vi "PicoScope4000ExampleBlock.vi"() -> ()   [LabVIEW 2012]
doc: "This example demonstrates how to use the PicoScope Labview library to collect data using block mode."
uses:
  shared/PicoBuffers.ctl
  shared/Acquisition Settings.ctl
  PicoScope4000Lib/PicoScope4000AnalogChannelSettingsIEPE.ctl
  PicoScope4000Lib/PicoScope4000Buffer and Transfer Settings.ctl
panel:
  in  "Channel B Settings":T1={"Enabled"=TRUE, "Range"=6, "Bandwidth Limit"=0, "Coupling"=1} {"Coupling" items=["AC", "DC", "IEPE"]; "Bandwidth Limit" items=["Off", "200kHz"]; "Range" items=["10 mV", "20 mV", "50 mV", "100 mV", "200 mV", "500 mV", "1 V", "2 V", "5 V", "10 V", "20 V", "50 V ", "100 V"]}
  out "Unit Info":T2
  in  "PicoScope 4262 Ext. Trigger Range":u32(ring)=5 items=["500 mV"=5, "5 V"=8]
  in  "Trigger Settings":T3={"Trigger Enabled"=FALSE, "Trigger Source"=enum."Channel A", "Trigger Threshold (Volts)"=0.0, "Trigger Direction"=2, "Trigger Delay (samples)"=0, "Auto Trigger Time (ms)"=1000} {"Trigger Direction" items=["Rising"=2, "Falling"=3]}
  in  "Channel A Settings":T1={"Enabled"=TRUE, "Range"=6, "Bandwidth Limit"=0, "Coupling"=1} {"Coupling" items=["AC", "DC", "IEPE"]; "Bandwidth Limit" items=["Off", "200kHz"]; "Range" items=["10 mV", "20 mV", "50 mV", "100 mV", "200 mV", "500 mV", "1 V", "2 V", "5 V", "10 V", "20 V", "50 V ", "100 V"]}
  out "overflow":i16 format="%08b"
  in  "Apply Settings":bool
  out "error out":errorcluster
  in  "Data file":path=path "PicoScope4000ExampleBlock ChA Data"
  in  "Buffer and Transfer Settings":T4={"startIndex"=0, "Samples"=5000000, "Down Sample Ratio"=1, "Down-Sample Mode"=0} {"Down-Sample Mode" items=["None", "Aggregate", "Average"]; "Down Sample Ratio" step=1; "Samples" format="%_6p"}
  in  "Acquisition Settings":T5={"preTriggerSamples"=0, "postTriggerSamples"=5000000, "timebase"=5} {"postTriggerSamples" format="%_6p"; "preTriggerSamples" format="%_6p"}
  out "Properties Panel":T6 {"Max Total Capture Time Available (sec)" format="%.3p"; "Sample Frequency" format="%.6p"; "Sample Rate" format="%.3p"; "Max Samples Available" format="%_6p"; "Total Capture Time (sec)" format="%.3p"}
  in  "stop":bool
  out "Analog Channels":cluster{i32, dbl, "Data":dbl[]}[](graph)
  in  "Serial Number":string
  in  "Use Serial Number":bool
  in  "error in (no error)":errorcluster
  # "Bit 0 = ChA"
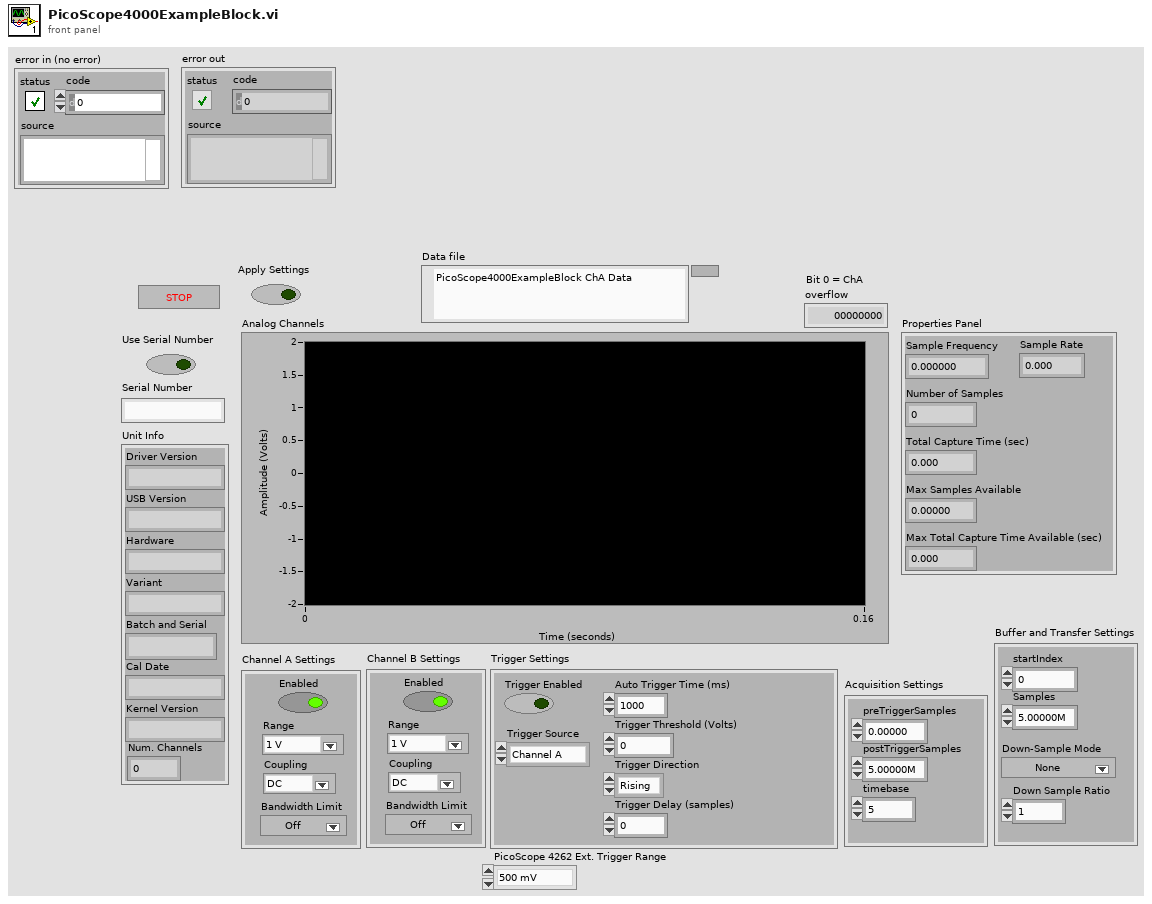
[diagram p1: front panel]
types:
  T1 = typedef "PicoScope4000AnalogChannelSettingsIEPE.ctl" = cluster{"Enabled":bool, "Range":u16, "Bandwidth Limit":i16, "Coupling":u16}
  T2 = cluster{"Driver Version":string, "USB Version":string, "Hardware":string, "Variant":string, "Batch and Serial":string, "Cal Date":string, "Kernel Version":string, "Num. Channels":i16}
  T3 = cluster{"Trigger Enabled":bool, "Trigger Source":enum16{"Channel A", "Channel B", "Channel C", "Channel D", "Channel E", "Channel F", "Channel G", "Channel H"}, "Trigger Threshold (Volts)":dbl, "Trigger Direction":u16, "Trigger Delay (samples)":u32, "Auto Trigger Time (ms)":i16}
  T4 = typedef "PicoScope4000Buffer and Transfer Settings.ctl" = cluster{"startIndex":u64, "Samples":u64, "Down Sample Ratio":u64, "Down-Sample Mode":u32}
  T5 = typedef "Acquisition Settings.ctl" = cluster{"preTriggerSamples":u64, "postTriggerSamples":u64, "timebase":u32}
  T6 = cluster{"Sample Frequency":dbl, "Sample Rate":dbl, "Max Samples Available":u64, "Number of Samples":u64, "Total Capture Time (sec) ":dbl, "Max Total Capture Time Available (sec)":dbl}
  T7 = enum16{"open", "open or create", "create or replace", "create", "open (read-only)"}
  T8 = typedef "PicoBuffers.ctl" = cluster{"Max Buffer Pointers":u64[][][], "Min Buffer Pointers":u64[][][], "StreamingDataInfo":cluster{"Channel":u32, "Down-Sample Mode":u32, "PICO_DATA_TYPE":enum32{"PICO_INT8_T", "PICO_INT16_T", "PICO_INT32_T", "PICO_UINT32_T", "PICO_INT64_T", ""}, "Samples":i32, "bufferIndex":u64, "startIndex":i32, "overflow":i16}[][]}
  T9 = cluster{"Channel A Buffer":i16[], "Channel B Buffer":i16[], "Channel C Buffer":i16[], "Channel D Buffer":i16[], "Channel E Buffer":i16[], "Channel F Buffer":i16[], "Channel G Buffer":i16[], "Channel H Buffer":i16[], "Port 0 Buffer":i16[], "Port 1 Buffer":i16[]}[]
  T10 = cluster{"Channel A Buffer":i16[], "Channel B Buffer":i16[], "Channel C Buffer":i16[], "Channel D Buffer":i16[], "Channel E Buffer":i16[], "Channel F Buffer":i16[], "Channel G Buffer":i16[], "Channel H Buffer":i16[], "Port 0 Buffer":i16[], "Port 1 Buffer":i16[]}
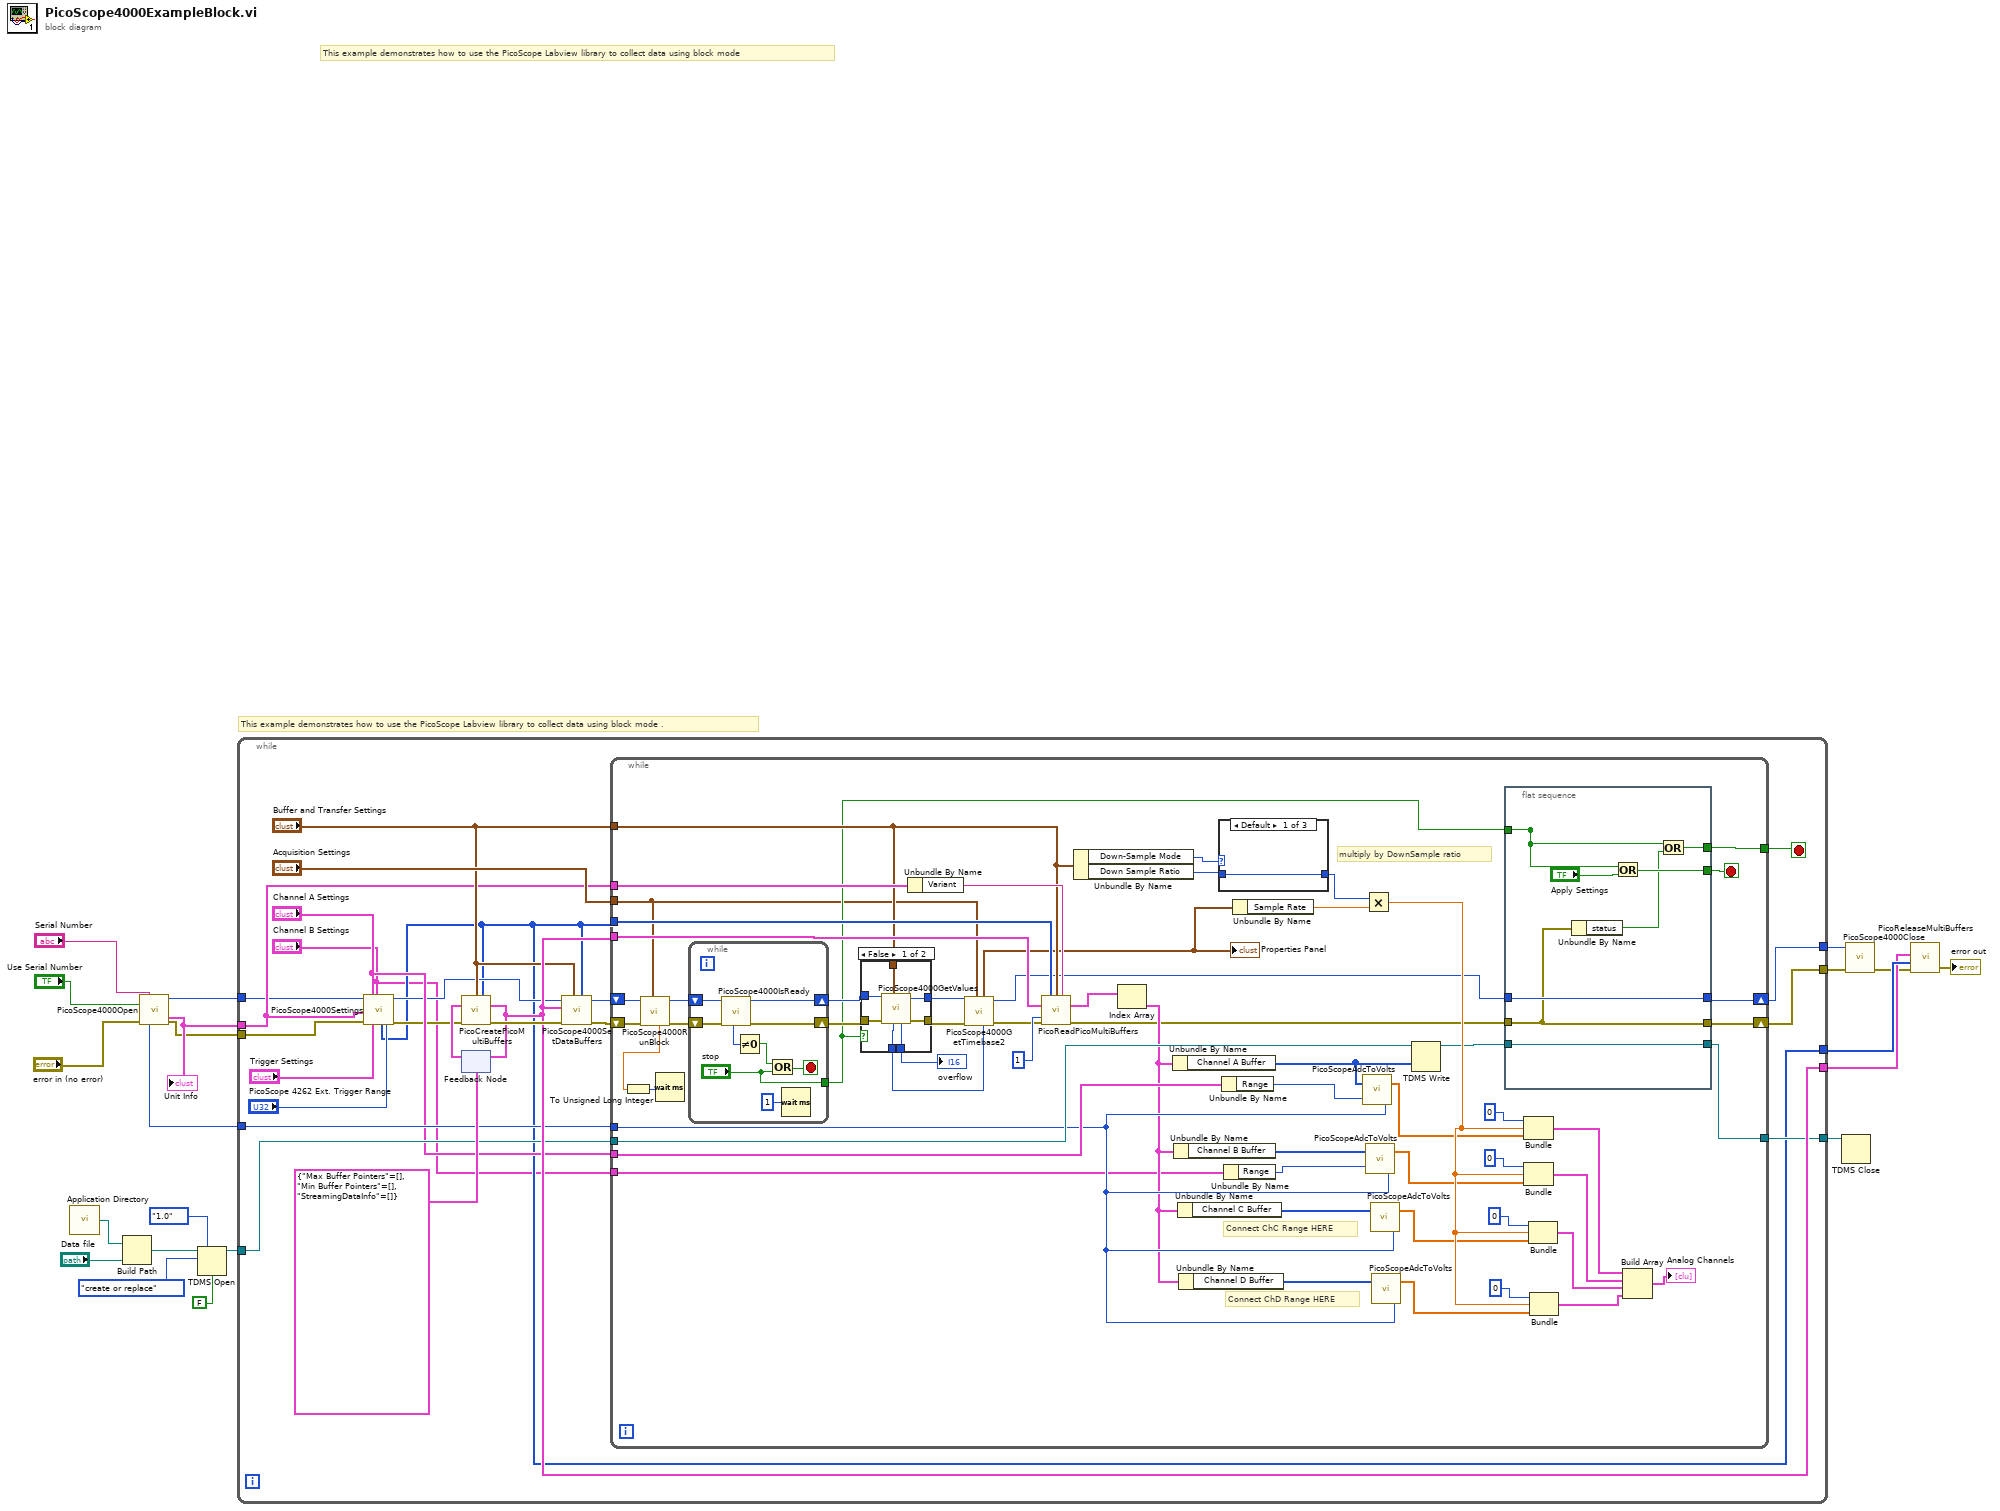
[diagram p0: block diagram]
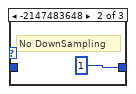
[diagram p3: hidden frame]
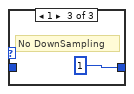
[diagram p4: hidden frame]
diagram:
  # "This example demonstrates how to use the PicoScope Labview library to collect data using block mode ."
  # "This example demonstrates how to use the PicoScope Labview library to collect data using block mode"
  n1 = call <vilib>:"Application Directory.vi"() -> ("Application Directory"=w14:path)
  n2 = Build Path(base path=w14, name or relative path="Data file") -> (appended path=w15:path)
  n3 = call "PicoScope4000Open.vi"("Serial Number"="Serial Number", "Use Serial Number"="Use Serial Number", "error in (no error)"="error in (no error)") -> ("handle"=w5:i16, "Max ADC value"=w10:i16, "Unit Info"=w6:T2, "error out"=w4:errorcluster)  [unwired: 9 in]
  "Unit Info" <- w6
  n4 = TDMS Open(6:FALSE ("disable buffering? (T)"), 7:enum16{"1.0", "2.0"}."1.0" ("file format version (2.0)"), 10:T7."create or replace" ("operation (0:open)"), 11:w15) -> (3:w12:refnum<k34>)  [unwired: 2 in, 1 out]
  n5 = while {
    tunnel: w10 -> [w39]
    tunnel: [w23] -> w21
    tunnel: [w42] -> w20
    tunnel: [w37] -> w13
    tunnel: w12 -> [w41]
    tunnel: [w38] -> w2
    tunnel: [w35] -> w9
    tunnel: w6 -> [w28]
    tunnel: w5 -> [w27]
    tunnel: w4 -> [w26]
    stop <- w36 stop-if-true
    n6 = call "PicoScope4000Settings.vi"("handle in"=w27, "Unit Info"=w28, "error in"=w26, "Channel A Settings"="Channel A Settings", "Trigger Settings"="Trigger Settings", "Channel B Settings"="Channel B Settings", "PicoScope 4262 Ext. Trigger Range"="PicoScope 4262 Ext. Trigger Range") -> ("Enabled array"=w23:i16[], "handle out"=w24:i16, "error out"=w25:errorcluster)  [unwired: 10 in]
    n7 = feedback #1(T8 {"Max Buffer Pointers"=[], "Min Buffer Pointers"=[], "StreamingDataInfo"=[]} ("Data Pointers")) -> (w44:T8)
    n8 = call "PicoCreatePicoMultiBuffers.vi"("Buffer and Transfer Settings"="Buffer and Transfer Settings", "enabled array"=w23, "Data Pointers In"=w44, "error in (no error)"=w25) -> ("Data Pointers"=w42:T8, "error out"=w43:errorcluster)  [unwired: 10 in]
    n9 = feedback-in #1(w42) -> ()
    n10 = call "PicoScope4000SetDataBuffers.vi"("enabled array"=w23, "Buffer and Transfer Settings"="Buffer and Transfer Settings", "error in (no error)"=w43, "Data Pointers In"=w42, "handle in"=w24) -> ("error out"=w34:errorcluster, "handle out"=w33:i16)  [unwired: 5 in]
    n11 = while {
      tunnel: w42 -> [w105]
      tunnel: "Buffer and Transfer Settings" -> [w59]
      tunnel: w23 -> [w96]
      tunnel: "Channel A Settings" -> [w95]
      tunnel: "Acquisition Settings" -> [w50]
      tunnel: w39 -> [w94]
      tunnel: w28 -> [w91]
      tunnel: [w66] -> w36
      shift-right: [w70] -> w38
      shift-left: w34 -> [w60]
      shift-right: [w64] -> w35
      shift-left: w33 -> [w61]
      tunnel: w41 -> [w104]
      tunnel: [w68] -> w37
      tunnel: "Channel B Settings" -> [w47]
      stop <- w65 stop-if-true
      # "Connect ChD Range HERE"
      # "Connect ChC Range HERE"
      # "multiply by DownSample ratio"
      n12 = call "PicoScope4000RunBlock.vi"("Acquisition Settings"=w50, "error in (no error)"=w60, "handle in"=w61) -> ("error out"=w98:errorcluster, "handle out"=w97:i16, "timeIndisposedMs"=w48:dbl)  [unwired: 5 in, 1 out]
      n13 = To Unsigned Long Integer(number=w48) -> (unsigned 32bit integer=w49:u32)
      n14 = Wait (ms)(milliseconds to wait=w49) -> ()  [unwired: 1 out]
      n15 = while {
        shift-right: [w130] -> w62
        shift-left: w98 -> [w131]
        shift-right: [w129] -> w63
        shift-left: w97 -> [w128]
        tunnel: ["stop"] -> w58
        stop <- w125 stop-if-true
        n16 = call "PicoScope4000IsReady.vi"("error in (no error)"=w131, "handle in"=w128) -> ("error out"=w130:errorcluster, "handle out"=w129:i16, "ready"=w127:i16)  [unwired: 7 in]
        n17 = Not Equal To 0?(x=w127) -> (x != 0?=w126:bool)
        n18 = Or(x=w126, y="stop") -> (x .or. y?=w125:bool)
        n19 = Wait (ms)(milliseconds to wait=u32 1) -> ()  [unwired: 1 out]
      }
      n20 = case shown="False" w58 {
        tunnel: w62 -> [w112 w113]
        tunnel: w63 -> [w111 w114]
        tunnel: [w110 w114] -> w52
        tunnel: [w109 w113] -> w53
        tunnel: w59 -> [w108 _]
        tunnel: [w107 _] -> w57
        tunnel: [w106 _] -> w56
        frame False {
          n21 = call "PicoScope4000GetValues.vi"("Buffer and Transfer Settings"=w108, "error in (no error)"=w112, "handle in"=w111) -> ("error out"=w109:errorcluster, "handle out"=w110:i16, "overflow"=w107:i16, "noOfSamples"=w106:u64)  [unwired: 5 in]
        }
        frame True {
        }
      }
      "overflow" <- w57
      n22 = Unbundle By Name(w91) -> ("Variant"=w92:string)
      n23 = call "PicoScope4000GetTimebase2.vi"("Number of Samples"=w56, "Acquisition Settings"=w50, "error in (no error)"=w53, "handle in"=w52) -> ("error out"=w54:errorcluster, "handle out"=w51:i16, "Properties Panel"=w55:T6)  [unwired: 5 in]
      "Properties Panel" <- w55
      n24 = call "PicoReadPicoMultiBuffers.vi"("enabled array"=w96, "Buffer and Transfer Settings"=w59, "Variant"=w92, "Data Pointers"=w105, "No of Buffers"=1, "error in (no error)"=w54) -> ("MultiBuffers (Max or non-aggregated)"=w103:T9, "error out"=w67:errorcluster)  [unwired: 7 in, 1 out]
      n25 = Unbundle By Name(w59) -> ("Down-Sample Mode"=w101:u32, "Down Sample Ratio"=w102:u64)
      n26 = Index Array(array=w103) -> (element=w71:T10)  [unwired: 1 in]
      n27 = Unbundle By Name(w71) -> ("Channel A Buffer"=w80:i16[])
      n28 = Unbundle By Name(w71) -> ("Channel B Buffer"=w86:i16[])
      n29 = Unbundle By Name(w71) -> ("Channel C Buffer"=w78:i16[])
      n30 = Unbundle By Name(w71) -> ("Channel D Buffer"=w74:i16[])
      n31 = case shown="Default" w101 {
        tunnel: [w132 u64 1 ("Down Sample Ratio") u64 1 ("Down Sample Ratio")] -> w99
        tunnel: w102 -> [w132 _ _]
        frame Default {
        }
        frame -2147483648 {
          # "No DownSampling"
        }
        frame 1 {
          # "No DownSampling"
        }
      }
      n32 = Unbundle By Name(w95) -> ("Range"=w88:u16)
      n33 = Unbundle By Name(w47) -> ("Range"=w46:u16)
      n34 = Unbundle By Name(w55) -> ("Sample Rate"=w93:dbl)
      n35 = call "PicoScopeAdcToVolts.vi"("Max_adc"=w94, "Range Index"=w88, "Data"=w80) -> ("Data"=w81:dbl[])
      n36 = Multiply(x=w99, y=w93) -> (x*y=w100:dbl)
      n37 = call "PicoScopeAdcToVolts.vi"("Max_adc"=w94, "Range Index"=w46, "Data"=w86) -> ("Data"=w85:dbl[])
      n38 = call "PicoScopeAdcToVolts.vi"("Max_adc"=w94, "Data"=w78) -> ("Data"=w77:dbl[])  [unwired: 1 in]
      n39 = call "PicoScopeAdcToVolts.vi"("Max_adc"=w94, "Data"=w74) -> ("Data"=w73:dbl[])  [unwired: 1 in]
      n40 = TDMS Write(0:w104, 9:w80) -> (4:w69:refnum<k34>)  [unwired: 4 in, 3 out]
      n41 = flat-sequence {
        tunnel: [w122] -> w65
        tunnel: [w115] -> _
        tunnel: [w119] -> w66
        tunnel: w51 -> [w118]
        tunnel: [w118] -> w64
        tunnel: w67 -> [w117]
        tunnel: [w117] -> w70
        tunnel: [w116] -> w68
        tunnel: w69 -> [w116]
        tunnel: w58 -> [w115]
        frame #0 {
          n42 = Unbundle By Name(w117) -> ("status"=w120:bool)
          n43 = Or(x=w115, y="Apply Settings") -> (x .or. y?=w122:bool)
          n44 = Or(x=w115, y=w120) -> (x .or. y?=w119:bool)
        }
      }
      n45 = Bundle(0, w100, "Data"=w81) -> (w84:cluster{i32, dbl, "Data":dbl[]})  [unwired: 1 in]
      n46 = Bundle(0, w100, "Data"=w85) -> (w83:cluster{i32, dbl, "Data":dbl[]})  [unwired: 1 in]
      n47 = Bundle(0, w100, "Data"=w77) -> (w76:cluster{i32, dbl, "Data":dbl[]})  [unwired: 1 in]
      n48 = Bundle(0, w100, "Data"=w73) -> (w72:cluster{i32, dbl, "Data":dbl[]})  [unwired: 1 in]
      n49 = Build Array(w84, w83, w76, w72) -> (→"Analog Channels":cluster{i32, dbl, "Data":dbl[]}[])
    }
  }
  n50 = TDMS Close(11:w13) -> ()  [unwired: 1 in, 2 out]
  n51 = call "PicoScope4000Close.vi"("error in (no error)"=w2, "handle"=w9) -> ("error out"=w1:errorcluster)  [unwired: 9 in]
  n52 = call "PicoReleaseMultiBuffers.vi"("error in (no error)"=w1, "Enabled array"=w21, "Data Pointers"=w20) -> ("error out"=→"error out":errorcluster)  [unwired: 8 in]
